vi "Write Boolean Output.vi"(8 "error in (no error)":errorcluster, 9 "Value":bool, 10 "Boolean Output":T1, 11 "Modbus in":refnum<class "Modbus.lvclass">) -> (0 "error out":errorcluster, 3 "Modbus out":refnum<class "Modbus.lvclass">)   [LabVIEW 2026, in "Modbus.lvlib" / "Modbus.lvclass"]
uses:
  Modbus.lvclass
  Types/Boolean Data.ctl
  Types/Modbus Table.ctl
  Modbus.lvclass/Modbus.ctl
  <vilib>/ni/Modbus Library/API/Master/Modbus Master.lvclass
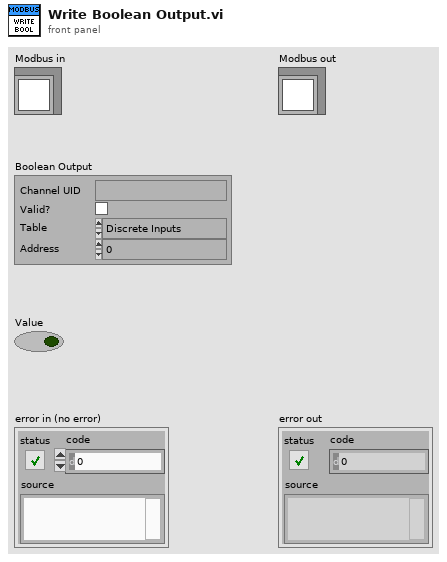
[diagram p1: front panel]
types:
  T1 = typedef "Modbus.lvlib/Modbus.lvclass/Boolean Data.ctl" = cluster{"Channel UID":string, "Valid?":bool, "Table":T2, "Address":i32}
  T2 = typedef "Modbus.lvlib/Modbus.lvclass/Modbus Table.ctl" = enum16{"Discrete Inputs", "Coils", "Input Registers", "Holding Registers"}
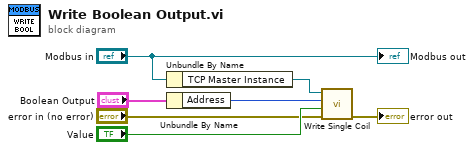
[diagram p0: block diagram]
diagram:
  n1 = Unbundle By Name("Modbus in") -> ("TCP Master Instance"=w2:refnum<class "Modbus Master.lvclass">)
  n2 = Unbundle By Name("Boolean Output") -> ("Address"=w1:i32)
  n3 = call-dynamic "Write Single Coil.vi"("error in"="error in (no error)", "coil to write"="Value", "address"=w1, "Modbus master in"=w2) -> ("error out"=→"error out":errorcluster)  [unwired: 6 in, 1 out]
  "Modbus out" <- "Modbus in"
